vi "ZM-TST-packages.vi"() -> (0 "error out":errorcluster, 3 "Pass":bool)   [LabVIEW 2020, in "ZM-TST-tests.lvlib"]
doc: "T1, round-trip test of the package classes: creates a test package, an error package and a bare package and checks their JSON, type names, destinations and timestamps against the typedefs. Pass = AND of the ten checks. Every error chain ends in error out."
uses:
  ZM-TST-tests.lvlib
  common/ZM-PC-packages/ZM-PC-package/ZM-PC-package.lvclass
  common/ZM-PC-packages/ZM-PC-TP-test_package/ZM-PC-TP-test_package.lvclass
  common/ZM-PC-packages/ZM-PC-EP-error_package/ZM-PC-EP-error_package.lvclass
panel:
  out "ep_root_ok":bool
  out "destination_roundtrip_ok":bool
  out "destination_default_ok":bool
  out "timestamp_ok":bool
  out "parent_json_ok":bool
  out "ep_json_ok":bool
  out "type_name_ok":bool
  out "tp_json_ok":bool
  out "call_parent_ok":bool
  out "dispatch_ok":bool
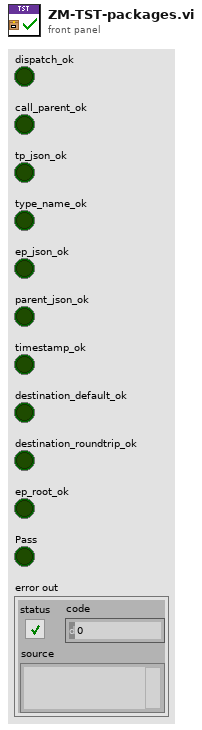
[diagram p1: front panel]
types:
  T1 = enum16{"Unknown", "Root", "Hardware", "Communication"}
  T2 = cluster{"timestamp":string, "type":string, "destination":string}
  T3 = cluster{"timestamp":string, "type":string, "destination":string, "data":cluster{"sender":string, "code":i32, "source":string}}
  T4 = cluster{"timestamp":string, "type":string, "destination":string, "data":cluster{"temperature_c":dbl, "sample_index":i32, "duty_percent":u8, "sensor_ok":bool, "status":string}}
  T5 = cluster{"temperature_c":dbl, "sample_index":i32, "duty_percent":u8, "sensor_ok":bool, "status":string}
  T6 = typedef "ZM-PC-packages.lvlib/ZM-PC-package.lvclass/ZM-PC-DESTINATION.ctl" = enum16{"Unknown", "Root", "Hardware", "Communication"}
  T7 = cluster{"temperature_c":bool, "sample_index":bool, "duty_percent":bool, "sensor_ok":bool, "status":bool}
  T8 = cluster{"sender":string, "code":i32, "source":string}
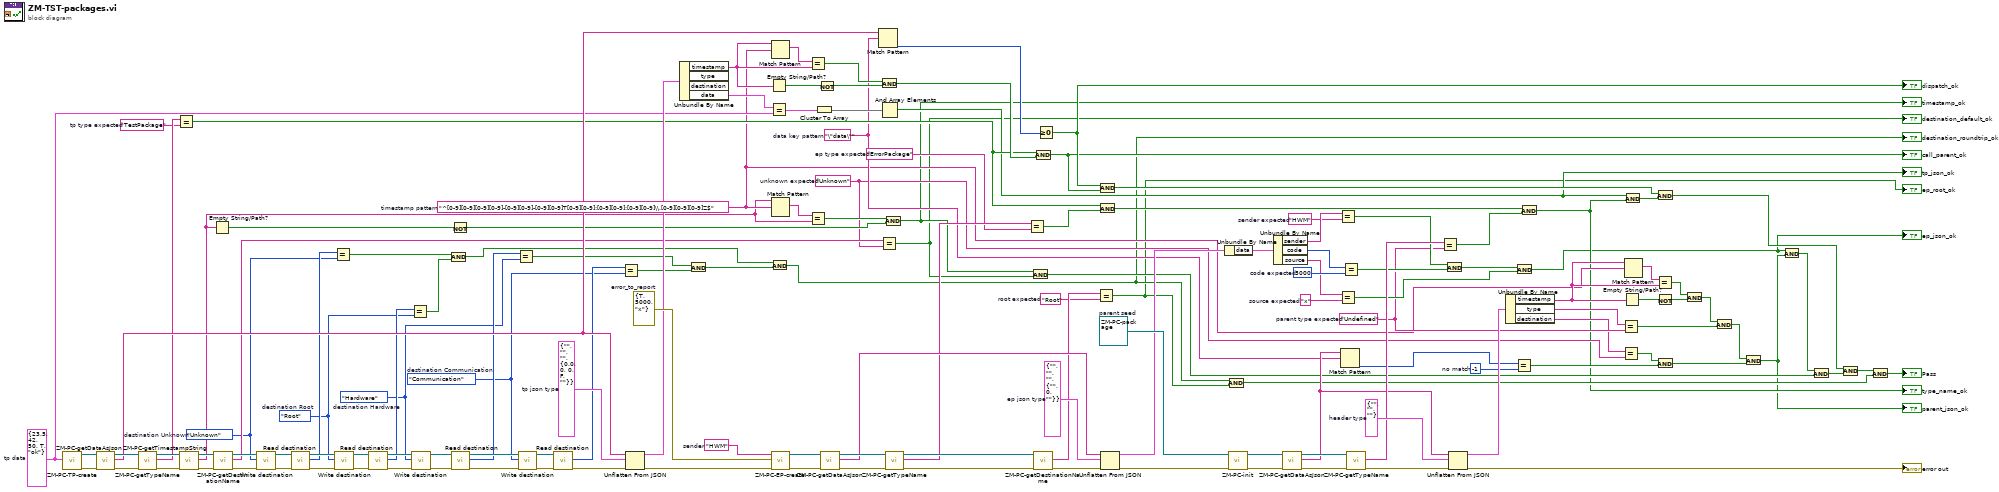
[diagram p0: block diagram]
diagram:
  w29 = T1."Communication"  # destination Communication
  w31 = T1."Hardware"  # destination Hardware
  w33 = T1."Root"  # destination Root
  w35 = T1."Unknown"  # destination Unknown
  w51 = -1  # no match
  w99 = T2 {"timestamp"="", "type"="", "destination"=""}  # header type
  w107 = T3 {"timestamp"="", "type"="", "destination"="", "data"={"sender"="", "code"=0, "source"=""}}  # ep json type
  w119 = T4 {"timestamp"="", "type"="", "destination"="", "data"={"temperature_c"=0.0, "sample_index"=0, "duty_percent"=0, "sensor_ok"=FALSE, "status"=""}}  # tp json type
  w68 = "x"  # source expected
  w70 = 5000  # code expected
  w72 = "HWM"  # sender expected
  w21 = "Root"  # root expected
  w37 = "Unknown"  # unknown expected
  w56 = "Undefined"  # parent type expected
  w81 = "ErrorPackage"  # ep type expected
  w94 = "TestPackage"  # tp type expected
  w53 = "\"data\""  # data key pattern
  w44 = "^[0-9][0-9][0-9][0-9]-[0-9][0-9]-[0-9][0-9]T[0-9][0-9]:[0-9][0-9]:[0-9][0-9]\\.[0-9][0-9][0-9]Z$"  # timestamp pattern
  w105 = refnum<class "ZM-PC-package.lvclass"> refnum  # parent seed
  w116 = errorcluster {"status"=TRUE, "code"=5000, "source"="x"}  # error_to_report
  w117 = "HWM"  # sender
  w85 = T5 {"temperature_c"=23.5, "sample_index"=42, "duty_percent"=50, "sensor_ok"=TRUE, "status"="ok"}  # tp data
  n1 = call "ZM-PC-TP-create.vi"("data"=w85) -> ("error out"=w142:errorcluster, "package"=w143:refnum<class "ZM-PC-TP-test_package.lvclass">)  [unwired: 9 in]
  n2 = call-dynamic "ZM-PC-getDataAsJson.vi"("error in (no error)"=w142, "ZM-PC-TP-test_package in"=w143) -> ("error out"=w140:errorcluster, "json"=w97:string, "ZM-PC-TP-test_package out"=w141:refnum<class "ZM-PC-TP-test_package.lvclass">)  [unwired: 7 in]
  n3 = call "ZM-PC-getTypeName.vi"("error in (no error)"=w140, "ZM-PC-package in"=w141) -> ("error out"=w138:errorcluster, "type_name"=w95:string, "ZM-PC-package out"=w139:refnum<class "ZM-PC-TP-test_package.lvclass">)  [unwired: 7 in]
  n4 = Equal?(x=w95, y=w94) -> (x = y?=w79:bool)
  n5 = call "ZM-PC-getTimestampString.vi"("error in (no error)"=w138, "ZM-PC-package in"=w139) -> ("error out"=w136:errorcluster, "timestamp_iso"=w42:string, "ZM-PC-package out"=w137:refnum<class "ZM-PC-TP-test_package.lvclass">)  [unwired: 7 in]
  n6 = Empty String/Path?(string/path=w42) -> (empty?=w41:bool)
  n7 = call "ZM-PC-getDestinationName.vi"("error in (no error)"=w136, "ZM-PC-package in"=w137) -> ("error out"=w135:errorcluster, "destination_name"=w38:string, "ZM-PC-package out"=w134:refnum<class "ZM-PC-TP-test_package.lvclass">)  [unwired: 7 in]
  n8 = call "Write destination.vi"("error in (no error)"=w135, "ZM-PC-DESTINATION"=w35, "ZM-PC-package in"=w134) -> ("error out"=w133:errorcluster, "ZM-PC-package out"=w132:refnum<class "ZM-PC-TP-test_package.lvclass">)  [unwired: 7 in]
  n9 = call "Read destination.vi"("error in (no error)"=w133, "ZM-PC-package in"=w132) -> ("error out"=w131:errorcluster, "ZM-PC-DESTINATION"=w36:T6, "ZM-PC-package out"=w130:refnum<class "ZM-PC-TP-test_package.lvclass">)  [unwired: 7 in]
  n10 = Equal?(x=w36, y=w35) -> (x = y?=w28:bool)
  n11 = call "Write destination.vi"("error in (no error)"=w131, "ZM-PC-DESTINATION"=w33, "ZM-PC-package in"=w130) -> ("error out"=w129:errorcluster, "ZM-PC-package out"=w128:refnum<class "ZM-PC-TP-test_package.lvclass">)  [unwired: 7 in]
  n12 = call "Read destination.vi"("error in (no error)"=w129, "ZM-PC-package in"=w128) -> ("error out"=w127:errorcluster, "ZM-PC-DESTINATION"=w34:T6, "ZM-PC-package out"=w126:refnum<class "ZM-PC-TP-test_package.lvclass">)  [unwired: 7 in]
  n13 = Equal?(x=w34, y=w33) -> (x = y?=w27:bool)
  n14 = call "Write destination.vi"("error in (no error)"=w127, "ZM-PC-DESTINATION"=w31, "ZM-PC-package in"=w126) -> ("error out"=w125:errorcluster, "ZM-PC-package out"=w124:refnum<class "ZM-PC-TP-test_package.lvclass">)  [unwired: 7 in]
  n15 = And(x=w28, y=w27) -> (x .and. y?=w24:bool)
  n16 = Not(x=w41) -> (.not. x?=w39:bool)
  n17 = call "Read destination.vi"("error in (no error)"=w125, "ZM-PC-package in"=w124) -> ("error out"=w123:errorcluster, "ZM-PC-DESTINATION"=w32:T6, "ZM-PC-package out"=w122:refnum<class "ZM-PC-TP-test_package.lvclass">)  [unwired: 7 in]
  n18 = Equal?(x=w32, y=w31) -> (x = y?=w26:bool)
  n19 = call "Write destination.vi"("error in (no error)"=w123, "ZM-PC-DESTINATION"=w29, "ZM-PC-package in"=w122) -> ("error out"=w121:errorcluster, "ZM-PC-package out"=w120:refnum<class "ZM-PC-TP-test_package.lvclass">)  [unwired: 7 in]
  n20 = call "Read destination.vi"("error in (no error)"=w121, "ZM-PC-package in"=w120) -> ("error out"=w118:errorcluster, "ZM-PC-DESTINATION"=w30:T6)  [unwired: 7 in, 1 out]
  n21 = Equal?(x=w30, y=w29) -> (x = y?=w25:bool)
  n22 = Unflatten From JSON(JSON string=w97, type and defaults=w119, error in (no error)=w118) -> (value=w93:T4, error out=w115:errorcluster)  [unwired: 4 in]
  n23 = Unbundle By Name(w93) -> ("timestamp"=w91:string, "data"=w86:T5)  [unwired: 2 out]
  n24 = And(x=w26, y=w25) -> (x .and. y?=w23:bool)
  n25 = Empty String/Path?(string/path=w91) -> (empty?=w90:bool)
  n26 = Equal?(x=w86, y=w85) -> (x = y?=w84:T7)
  n27 = And(x=w24, y=w23) -> (x .and. y?=w4:bool)
  "destination_roundtrip_ok" <- w4
  n28 = Match Pattern(string=w91, regular expression=w44) -> (match substring=w92:string)  [unwired: 1 in, 3 out]
  n29 = Match Pattern(string=w42, regular expression=w44) -> (match substring=w43:string)  [unwired: 1 in, 3 out]
  n30 = call "ZM-PC-EP-create.vi"("error in (no error)"=w115, "error_to_report"=w116, "sender"=w117) -> ("error out"=w113:errorcluster, "package"=w114:refnum<class "ZM-PC-EP-error_package.lvclass">)  [unwired: 7 in]
  n31 = Equal?(x=w92, y=w91) -> (x = y?=w89:bool)
  n32 = Equal?(x=w43, y=w42) -> (x = y?=w40:bool)
  n33 = Cluster To Array(cluster=w84) -> (array=w83:bool[])
  n34 = Not(x=w90) -> (.not. x?=w88:bool)
  n35 = call-dynamic "ZM-PC-getDataAsJson.vi"("error in (no error)"=w113, "ZM-PC-EP-error_package in"=w114) -> ("error out"=w111:errorcluster, "json"=w108:string, "ZM-PC-EP-error_package out"=w112:refnum<class "ZM-PC-EP-error_package.lvclass">)  [unwired: 7 in]
  n36 = Match Pattern(string=w97, regular expression=w53) -> (offset past match=w96:i32)  [unwired: 1 in, 3 out]
  n37 = Equal?(x=w38, y=w37) -> (x = y?=w5:bool)
  "destination_default_ok" <- w5
  n38 = And(x=w89, y=w88) -> (x .and. y?=w87:bool)
  n39 = And Array Elements(Boolean array=w83) -> (logical AND=w10:bool)
  "tp_json_ok" <- w10
  n40 = And(x=w40, y=w39) -> (x .and. y?=w6:bool)
  "timestamp_ok" <- w6
  n41 = call "ZM-PC-getTypeName.vi"("error in (no error)"=w111, "ZM-PC-package in"=w112) -> ("error out"=w109:errorcluster, "type_name"=w82:string, "ZM-PC-package out"=w110:refnum<class "ZM-PC-EP-error_package.lvclass">)  [unwired: 7 in]
  n42 = Equal?(x=w82, y=w81) -> (x = y?=w78:bool)
  n43 = And(x=w6, y=w5) -> (x .and. y?=w17:bool)
  n44 = call "ZM-PC-getDestinationName.vi"("error in (no error)"=w109, "ZM-PC-package in"=w110) -> ("error out"=w106:errorcluster, "destination_name"=w22:string)  [unwired: 7 in, 1 out]
  n45 = And(x=w79, y=w87) -> (x .and. y?=w11:bool)
  "call_parent_ok" <- w11
  n46 = Greater Or Equal To 0?(x=w96) -> (x >= 0?=w12:bool)
  "dispatch_ok" <- w12
  n47 = Equal?(x=w22, y=w21) -> (x = y?=w3:bool)
  "ep_root_ok" <- w3
  n48 = And(x=w12, y=w11) -> (x .and. y?=w20:bool)
  n49 = And(x=w79, y=w78) -> (x .and. y?=w77:bool)
  n50 = Unflatten From JSON(JSON string=w108, type and defaults=w107, error in (no error)=w106) -> (value=w75:T3, error out=w104:errorcluster)  [unwired: 4 in]
  n51 = Unbundle By Name(w75) -> ("data"=w74:T8)
  n52 = And(x=w4, y=w3) -> (x .and. y?=w13:bool)
  n53 = call-dynamic "ZM-PC-init.vi"("error in (no error)"=w104, "ZM-PC-package in"=w105) -> ("error out"=w102:errorcluster, "ZM-PC-package out"=w103:refnum<class "ZM-PC-package.lvclass">)  [unwired: 8 in]
  n54 = Unbundle By Name(w74) -> ("sender"=w73:string, "code"=w71:i32, "source"=w69:string)
  n55 = call-dynamic "ZM-PC-getDataAsJson.vi"("error in (no error)"=w102, "ZM-PC-package in"=w103) -> ("error out"=w100:errorcluster, "json"=w54:string, "ZM-PC-package out"=w101:refnum<class "ZM-PC-package.lvclass">)  [unwired: 7 in]
  n56 = Equal?(x=w73, y=w72) -> (x = y?=w67:bool)
  n57 = Equal?(x=w69, y=w68) -> (x = y?=w64:bool)
  n58 = Match Pattern(string=w54, regular expression=w53) -> (offset past match=w52:i32)  [unwired: 1 in, 3 out]
  n59 = Equal?(x=w71, y=w70) -> (x = y?=w66:bool)
  n60 = call "ZM-PC-getTypeName.vi"("error in (no error)"=w100, "ZM-PC-package in"=w101) -> ("error out"=w98:errorcluster, "type_name"=w80:string)  [unwired: 7 in, 1 out]
  n61 = Equal?(x=w80, y=w56) -> (x = y?=w76:bool)
  n62 = And(x=w67, y=w66) -> (x .and. y?=w65:bool)
  n63 = Unflatten From JSON(JSON string=w54, type and defaults=w99, error in (no error)=w98) -> (value=w63:T2, error out=→"error out":errorcluster)  [unwired: 4 in]
  n64 = Unbundle By Name(w63) -> ("timestamp"=w61:string, "type"=w57:string, "destination"=w55:string)
  n65 = Equal?(x=w52, y=w51) -> (x = y?=w47:bool)
  n66 = And(x=w65, y=w64) -> (x .and. y?=w8:bool)
  "ep_json_ok" <- w8
  n67 = And(x=w77, y=w76) -> (x .and. y?=w9:bool)
  "type_name_ok" <- w9
  n68 = Equal?(x=w57, y=w56) -> (x = y?=w49:bool)
  n69 = Equal?(x=w55, y=w37) -> (x = y?=w48:bool)
  n70 = Empty String/Path?(string/path=w61) -> (empty?=w60:bool)
  n71 = And(x=w10, y=w9) -> (x .and. y?=w19:bool)
  n72 = Match Pattern(string=w61, regular expression=w44) -> (match substring=w62:string)  [unwired: 1 in, 3 out]
  n73 = Equal?(x=w62, y=w61) -> (x = y?=w59:bool)
  n74 = Not(x=w60) -> (.not. x?=w58:bool)
  n75 = And(x=w20, y=w19) -> (x .and. y?=w16:bool)
  n76 = And(x=w48, y=w47) -> (x .and. y?=w45:bool)
  n77 = And(x=w59, y=w58) -> (x .and. y?=w50:bool)
  n78 = And(x=w50, y=w49) -> (x .and. y?=w46:bool)
  n79 = And(x=w46, y=w45) -> (x .and. y?=w7:bool)
  "parent_json_ok" <- w7
  n80 = And(x=w8, y=w7) -> (x .and. y?=w18:bool)
  n81 = And(x=w18, y=w17) -> (x .and. y?=w15:bool)
  n82 = And(x=w16, y=w15) -> (x .and. y?=w14:bool)
  n83 = And(x=w14, y=w13) -> (x .and. y?=→"Pass":bool)
